vi "test24-MappingRelationshipByExternalRegistration_API.vi"(8 "error in (no error)":errorcluster, 11 "TestCase in":refnum<class "testcase-CSMBroadcast.lvclass">) -> (0 "error out":errorcluster, 3 "TestCase out":refnum<class "testcase-CSMBroadcast.lvclass">)   [LabVIEW 2017, in "testcase-CSMBroadcast.lvclass"]
uses:
  testcase-CSMBroadcast.lvclass
  src/user.lib/_NEVSTOP/Communicable State Machine(CSM)/Communicable State Machine.lvlib
  <vilib>/addons/_JKI Toolkits/VI Tester/TestCase.llb/TestCase.lvclass
  C:/Program Files (x86)/National Instruments/LabVIEW 2017/vi.lib/addons/_JKI Toolkits/VI Tester/TestCase.llb/TestCase.lvclass
panel:
  out "Loop Count":i32
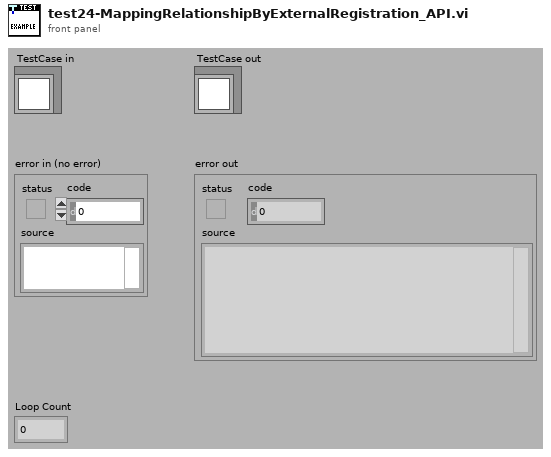
[diagram p1: front panel]
types:
  T1 = cluster{"Status":string, "Source CSM":string, "Target CSM":string, "Target API":string}[]
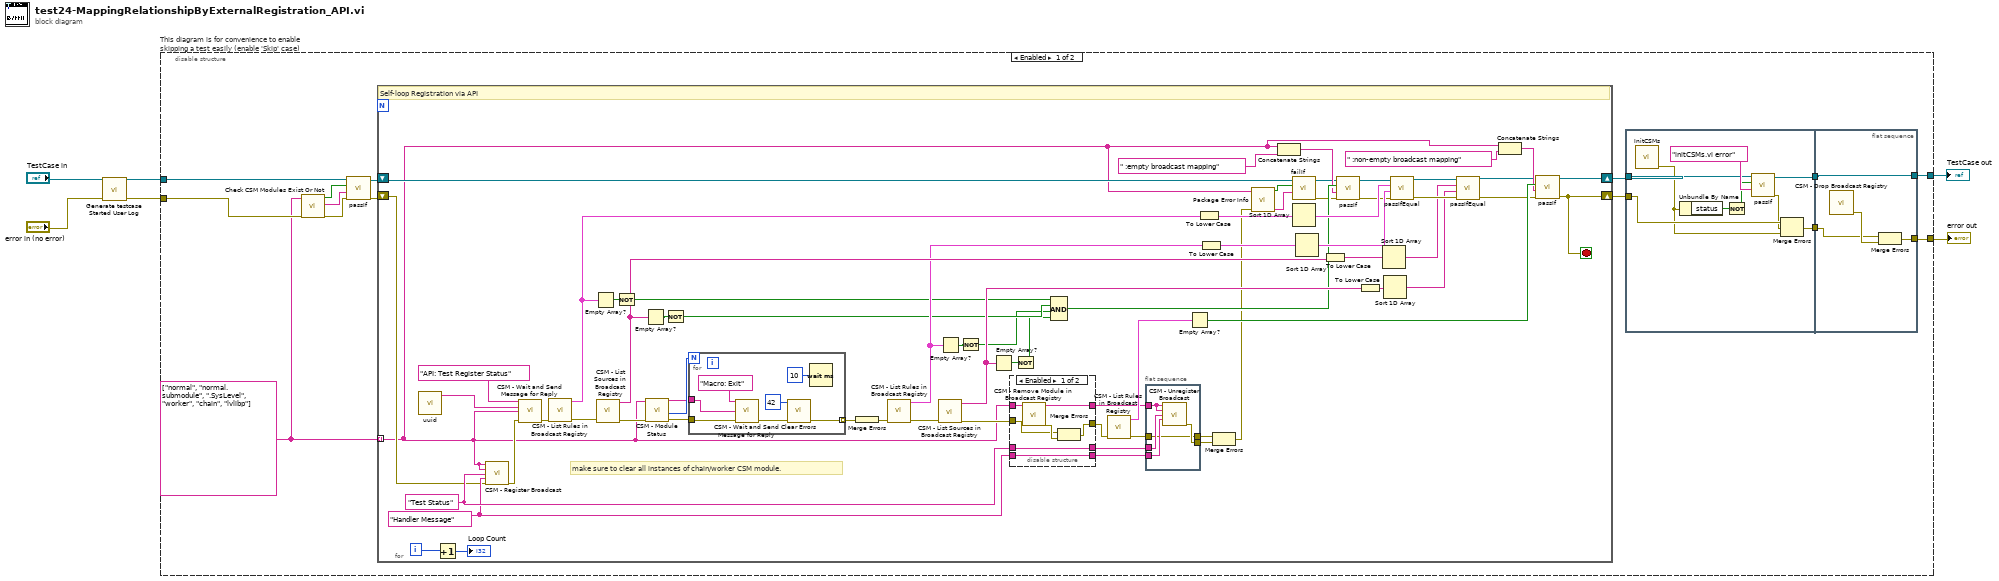
[diagram p0: block diagram]
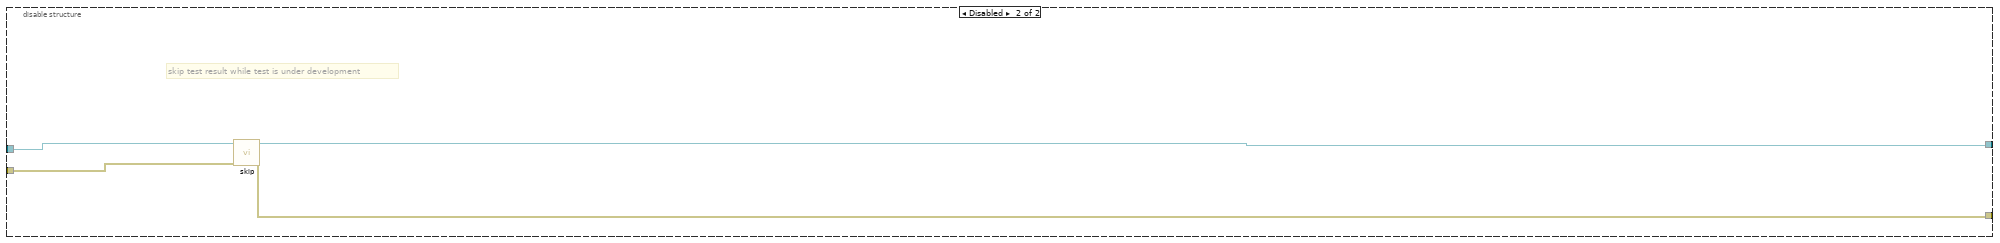
[diagram p3: hidden frame]
diagram:
  n1 = call "Generate testcase Started User Log.vi"("Error In"="error in (no error)") -> ("error out"=w1:errorcluster)  [unwired: 10 in]
  n2 = disable-structure "This diagram is for convenience to enable skipping a test easily (enable 'Skip' case)" shown="Enabled" {
    disable-tunnel: "TestCase in" -> [w13 w126]
    disable-tunnel: [w8 w124] -> w2
    disable-tunnel: [w7 w125] -> w4
    disable-tunnel: w1 -> [w11 w123]
    frame Enabled {
      w9 = string[] ["normal", "normal.submodule", ".SysLevel", "worker", "chain", "lvlibp"]
      n3 = call "Check CSM Modules Exist Or Not.vi"("error in"=w11, "CSM names in"=w9) -> ("error out"=w14:errorcluster, "Debug string"=w15:string, "All Modules Exist?"=w16:bool)  [unwired: 7 in]
      n4 = call-dynamic "passIf.vi"("error in (no error)"=w14, "message (\"\")"=w15, "pass"=w16, "TestCase in"=w13) -> ("error out"=w10:errorcluster, "TestCase out"=w12:refnum<class "testcase-CSMBroadcast.lvclass">)  [unwired: 6 in]
      n5 = for {
        tunnel: w9 -> [w41] mode=indexing
        shift-right: [w65] -> w18
        shift-left: w12 -> [w44]
        shift-right: [w63] -> w17
        shift-left: w10 -> [w51]
        i -> [w84]
        stop <- w63 stop-if-true
        w67 = "Handler Message" ("Response Message (If \"\", Same as Source Message)")
        w68 = "Test Status" ("Status")
        # "make sure to clear all instances of chain/worker CSM module."
        # "Self-loop Registration via API"
        n6 = call "uuid.vi"() -> ("UUID"=w98:string)  [unwired: 11 in]
        n7 = Increment(x=w84) -> (x+1=→"Loop Count":i32)
        n8 = call "CSM - Register Broadcast.vi"("CSM Name(Empty for Broadcast Event)"=w41, "Source CSM Name (* as Default)"=w41, "Trigger"=w68, "API (If \"\", Same as Trigger)"=w67, "Error In"=w51) -> ("error out"=w69:errorcluster)  [unwired: 9 in, 1 out]
        n9 = call "CSM - Wait and Send Message for Reply.vi"("State"="API: Test Register Status", "Arguments (\"\")"=w98, "Target Module"=w41, "Error In (No Error)"=w69) -> ("error out"=w97:errorcluster)  [unwired: 8 in, 3 out]
        n10 = call "CSM - List Rules in Broadcast Registry.vi"("error in (no error)"=w97) -> ("error out"=w96:errorcluster, "Rule Entries"=w82:T1)  [unwired: 8 in, 1 out]
        n11 = Empty Array?(array=w82) -> (empty?=w81:bool)
        n12 = call "CSM - List Sources in Broadcast Registry.vi"("error in (no error)"=w96) -> ("error out"=w60:errorcluster, "Broadcast Names"=w79:string[])  [unwired: 9 in]
        n13 = Not(x=w81) -> (.not. x?=w74:bool)
        n14 = Empty Array?(array=w79) -> (empty?=w80:bool)
        n15 = call "CSM - Module Status.vi"("Error In"=w60, "CSM Name"=w41) -> ("error out"=w59:errorcluster, "#Nodes"=w62:i32, "CSM Name (Dup)"=w61:string)  [unwired: 5 in, 2 out]
        n16 = Not(x=w80) -> (.not. x?=w73:bool)
        n17 = for {
          N: w62 -> [_]
          tunnel: w61 -> [w110]
          tunnel: w59 -> [w109]
          tunnel: [w107] -> w57 mode=indexing
          n18 = call "CSM - Wait and Send Message for Reply.vi"("State"="Macro: Exit", "Target Module"=w110, "Error In (No Error)"=w109) -> ("error out"=w108:errorcluster)  [unwired: 9 in, 3 out]
          n19 = call <vilib>:"Clear Errors.vi"("error in (no error)"=w108, "specific error code to clear (0: all)"=42) -> ("error out"=w107:errorcluster)  [unwired: 4 in, 1 out]
          n20 = Wait (ms)(milliseconds to wait=u32 10) -> ()  [unwired: 1 out]
        }
        n21 = Merge Errors(w57) -> (w58:errorcluster)
        n22 = call "CSM - List Rules in Broadcast Registry.vi"("error in (no error)"=w58) -> ("error out"=w95:errorcluster, "Rule Entries"=w77:T1)  [unwired: 8 in, 1 out]
        n23 = call "CSM - List Sources in Broadcast Registry.vi"("error in (no error)"=w95) -> ("error out"=w70:errorcluster, "Broadcast Names"=w75:string[])  [unwired: 9 in]
        n24 = Empty Array?(array=w77) -> (empty?=w78:bool)
        n25 = Not(x=w78) -> (.not. x?=w72:bool)
        n26 = Empty Array?(array=w75) -> (empty?=w76:bool)
        n27 = disable-structure shown="Enabled" {
          disable-tunnel: w70 -> [w112 w121]
          disable-tunnel: [w116 w121] -> w39
          disable-tunnel: w41 -> [w117 w122]
          disable-tunnel: w68 -> [w114 w120]
          disable-tunnel: w67 -> [w113 w119]
          disable-tunnel: [w115 w122] -> w40
          disable-tunnel: [w114 w120] -> w38
          disable-tunnel: [w113 w119] -> w37
          frame Enabled {
            n28 = call "CSM - Remove Module in Broadcast Registry.vi"("CSM Name"=w117) -> ("CSM Name (Dup)"=w115:string, "error out"=w118:errorcluster)  [unwired: 13 in]
            n29 = Merge Errors(w112, w118) -> (w116:errorcluster)
          }
          frame Disabled {
          }
        }
        n30 = Not(x=w76) -> (.not. x?=w71:bool)
        n31 = Compound Arithmetic op=AND(w74, w73, w72, w71) -> (w50:bool)
        n32 = call "CSM - List Rules in Broadcast Registry.vi"("error in (no error)"=w39) -> ("error out"=w34:errorcluster, "Rule Entries"=w66:T1)  [unwired: 8 in, 1 out]
        n33 = flat-sequence {
          tunnel: w40 -> [w104]
          tunnel: w38 -> [w103]
          tunnel: w37 -> [w102]
          tunnel: [w101] -> w36
          tunnel: w34 -> [w100]
          tunnel: [w100] -> w33
          frame #0 {
            n34 = call "CSM - Unregister Broadcast.vi"("CSM Name(Empty for Broadcast Event)"=w104, "Source CSM Name (* as Default)"=w104, "Trigger"=w103, "API (\"*\" as Default)"=w102) -> ("error out"=w101:errorcluster)  [unwired: 10 in, 1 out]
          }
        }
        n35 = Empty Array?(array=w66) -> (empty?=w64:bool)
        n36 = To Lower Case(string=w82) -> (all lower case string=w94:T1)
        n37 = To Lower Case(string=w77) -> (all lower case string=w93:T1)
        n38 = Merge Errors(w33, w36) -> (w35:errorcluster)
        n39 = call "Package Error Info.vi"("error in"=w35, "String in"=w41) -> ("packed error info out"=w45:string, "error status"=w46:bool)  [unwired: 8 in]
        n40 = Concatenate Strings(w41, " :empty broadcast mapping" ("string")) -> (w49:string)
        n41 = call-dynamic "failIf.vi"("message (\"\")"=w45, "fail"=w46, "TestCase in"=w44) -> ("error out"=w42:errorcluster, "TestCase out"=w43:refnum<class "testcase-CSMBroadcast.lvclass">)  [unwired: 7 in]
        n42 = Sort 1D Array(array=w94) -> (sorted array=w92:T1)
        n43 = Sort 1D Array(array=w93) -> (sorted array=w91:T1)
        n44 = To Lower Case(string=w79) -> (all lower case string=w88:string[])
        n45 = call-dynamic "passIf.vi"("error in (no error)"=w42, "message (\"\")"=w49, "pass"=w50, "TestCase in"=w43) -> ("error out"=w53:errorcluster, "TestCase out"=w52:refnum<class "testcase-CSMBroadcast.lvclass">)  [unwired: 6 in]
        n46 = To Lower Case(string=w75) -> (all lower case string=w87:string[])
        n47 = Sort 1D Array(array=w88) -> (sorted array=w86:string[])
        n48 = Sort 1D Array(array=w87) -> (sorted array=w85:string[])
        n49 = call-dynamic "passIfEqual.vi"("error in (no error)"=w53, "y"=w91, "x"=w92, "TestCase in"=w52) -> ("error out"=w89:errorcluster, "TestCase out"=w90:refnum<class "testcase-CSMBroadcast.lvclass">)  [unwired: 6 in]
        n50 = call-dynamic "passIfEqual.vi"("error in (no error)"=w89, "y"=w85, "x"=w86, "TestCase in"=w90) -> ("error out"=w47:errorcluster, "TestCase out"=w48:refnum<class "testcase-CSMBroadcast.lvclass">)  [unwired: 6 in]
        n51 = Concatenate Strings(w41, " :non-empty broadcast mapping" ("string")) -> (w54:string)
        n52 = call-dynamic "passIf.vi"("error in (no error)"=w47, "message (\"\")"=w54, "pass"=w64, "TestCase in"=w48) -> ("error out"=w63:errorcluster, "TestCase out"=w65:refnum<class "testcase-CSMBroadcast.lvclass">)  [unwired: 6 in]
      }
      n53 = flat-sequence {
        tunnel: w18 -> [w20]
        tunnel: [w28] -> w19
        tunnel: w17 -> [w25]
        tunnel: [w22] -> w6
        tunnel: w19 -> [w31]
        tunnel: [w31] -> w8
        tunnel: [w30] -> w7
        tunnel: w6 -> [w29]
        frame #0 {
          n54 = call "InitCSMs.vi"() -> ("error out"=w23:errorcluster)  [unwired: 10 in, 1 out]
          n55 = Unbundle By Name(w23) -> ("status"=w27:bool)
          n56 = Not(x=w27) -> (.not. x?=w21:bool)
          n57 = call-dynamic "passIf.vi"("message (\"\")"="initCSMs.vi error" ("message (\"\")"), "pass"=w21, "TestCase in"=w20) -> ("error out"=w24:errorcluster, "TestCase out"=w28:refnum<class "testcase-CSMBroadcast.lvclass">)  [unwired: 7 in]
          n58 = Merge Errors(w25, w24, w23) -> (w22:errorcluster)
        }
        frame #1 {
          n59 = call "CSM - Drop Broadcast Registry.vi"() -> ("error out"=w32:errorcluster)  [unwired: 15 in]
          n60 = Merge Errors(w29, w32) -> (w30:errorcluster)
        }
      }
    }
    frame Disabled {
      # "skip test result while test is under development"
      n61 = call <vilib>:"skip.vi"("error in (no error)"=w123, "TestCase in"=w126) -> ("error out"=w125:errorcluster, "TestCase out"=w124:refnum<class "testcase-CSMBroadcast.lvclass">)  [unwired: 8 in]
    }
  }
  "error out" <- w4
  "TestCase out" <- w2
